vi "Add New State.vi"(7 "After State (Optional)":string, 8 "error in (no error)":errorcluster, 9 "State Name":string, 10 "Category (Optional)":string, 11 "JKI SM in":refnum<class "JKI SM.lvclass">) -> (0 "error out":errorcluster, 1 "New Frame Name":string, 3 "JKI SM out":refnum<class "JKI SM.lvclass">)   [LabVIEW 2020, in "JKI State Machine API.lvlib" / "JKI SM.lvclass"]
uses:
  JKI SM.lvclass
  JKI SM.lvclass/JKI SM.ctl
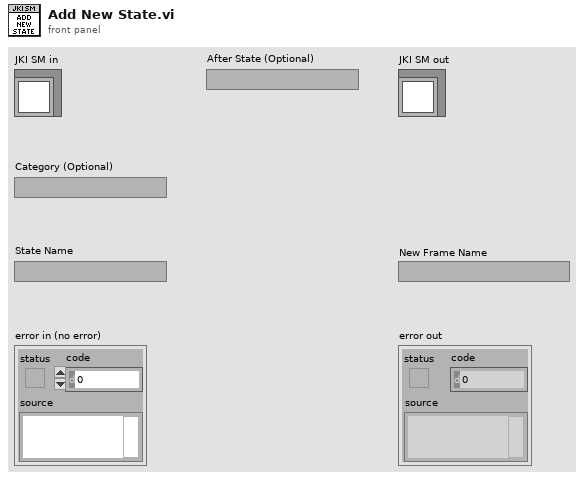
[diagram p1: front panel]
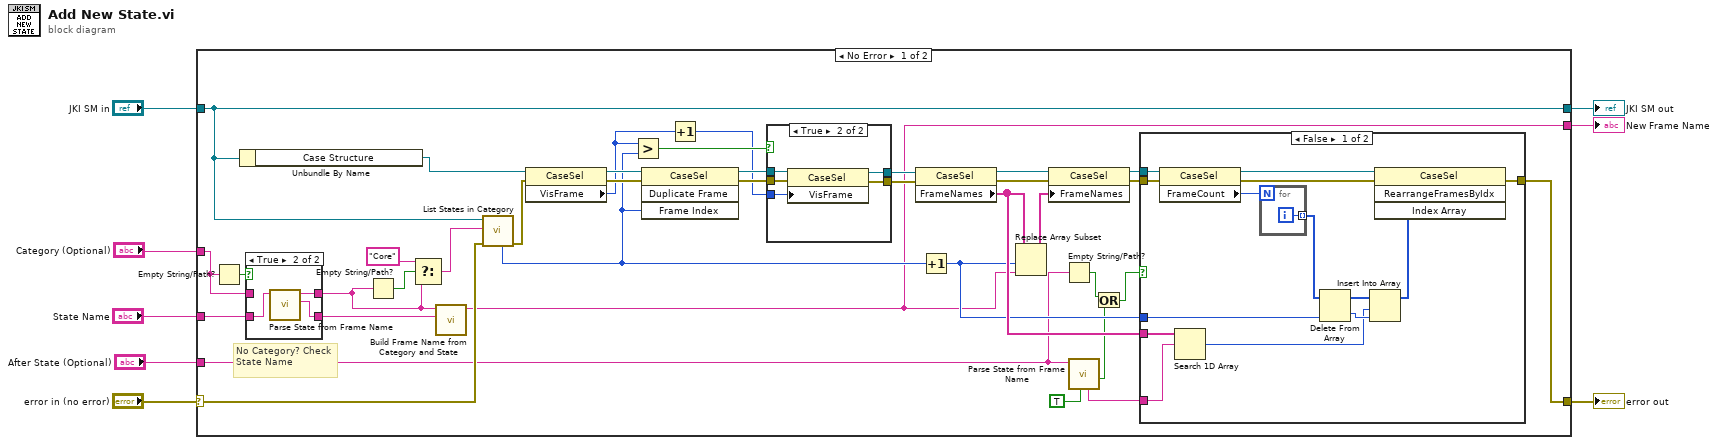
[diagram p0: block diagram]
diagram:
  n1 = case shown="No Error" "error in (no error)" {
    selector: "error in (no error)" -> [w42 w75]
    tunnel: [w16 w75] -> w7
    tunnel: [w20 w74] -> w5
    tunnel: "JKI SM in" -> [w20 w74]
    tunnel: "State Name" -> [w28 _]
    tunnel: "Category (Optional)" -> [w29 _]
    tunnel: "After State (Optional)" -> [w14 _]
    tunnel: [w9 _] -> w1
    frame No Error {
      # "No Category? Check State Name"
      n2 = Empty String/Path?(string/path=w29) -> (empty?=w30:bool)
      n3 = Unbundle By Name(w20) -> ("Case Structure"=w41:refnum<vi>)
      n4 = case shown="True" w30 {
        tunnel: w28 -> [w62 w66]
        tunnel: [w63 w65] -> w23
        tunnel: w29 -> [w63 _]
        tunnel: [w62 w64] -> w27
        frame False {
        }
        frame True {
          n5 = call "Parse State from Frame Name.vi"("Frame or State Name"=w66) -> ("State Name"=w64:string, "Category Name"=w65:string)  [unwired: 5 in, 4 out]
        }
      }
      n6 = Empty String/Path?(string/path=w23) -> (empty?=w25:bool)
      n7 = Select(t="Core" ("Category"), s=w25, f=w23) -> (s? t:f=w22:string)
      n8 = call "Build Frame Name from Category and State.vi"("State Name"=w27, "Category"=w23) -> ("Frame Name"=w9:string)  [unwired: 9 in]
      n9 = call "List States in Category.vi"("error in (no error)"=w42, "Category"=w22, "JKI SM in"=w20) -> ("error out"=w39:errorcluster, "Category Frame Index"=w26:i32)  [unwired: 4 in, 3 out]
      n10 = property class="CaseSel"(reference=w41, error in=w39) -> (reference out=w40:refnum<vi>, error out=w38:errorcluster, "VisFrame"=w33:u32)
      n11 = Greater?(x=w33, y=w26) -> (0:w32:bool)
      n12 = invoke class="CaseSel" method="Duplicate Frame"(reference=w40, error in=w38, "Frame Index"=w26) -> (reference out=w35:refnum<vi>, error out=w34:errorcluster)  [unwired: 1 in, 2 out]
      n13 = Increment(x=w33) -> (x+1=w31:u32)
      n14 = case shown="True" w32 {
        tunnel: [w68 w73] -> w37
        tunnel: [w67 w72] -> w36
        tunnel: w35 -> [w68 w71]
        tunnel: w34 -> [w67 w70]
        tunnel: w31 -> [_ w69]
        frame False {
        }
        frame True {
          n15 = property class="CaseSel"(reference=w71, error in=w70, "VisFrame"=w69) -> (reference out=w73:refnum<vi>, error out=w72:errorcluster)
        }
      }
      n16 = property class="CaseSel"(reference=w37, error in=w36) -> (reference out=w45:refnum<vi>, error out=w44:errorcluster, "FrameNames"=w21:string[])
      n17 = Increment(x=w26) -> (x+1=w18:i32)
      n18 = Replace Array Subset(array=w21, new element=w9, index=w18) -> (w43:string[])
      n19 = property class="CaseSel"(reference=w45, error in=w44, "FrameNames"=w43) -> (reference out=w19:refnum<vi>, error out=w17:errorcluster)
      n20 = Empty String/Path?(string/path=w14) -> (empty?=w12:bool)
      n21 = call "Parse State from Frame Name.vi"("Wrap in Quotes? (FALSE)"=TRUE, "Frame or State Name"=w14) -> ("is a Category Frame?"=w13:bool, "\"Category: State\" String"=w10:string)  [unwired: 4 in, 4 out]
      n22 = Or(x=w12, y=w13) -> (x .or. y?=w11:bool)
      n23 = case shown="False" w11 {
        tunnel: w21 -> [w54 _]
        tunnel: w19 -> [w52 _]
        tunnel: w18 -> [w51 _]
        tunnel: w17 -> [w48 w61]
        tunnel: [w49 w61] -> w16
        tunnel: w10 -> [w46 _]
        frame False {
          n24 = property class="CaseSel"(reference=w52, error in=w48) -> (reference out=w50:refnum<vi>, error out=w47:errorcluster, "FrameCount"=w55:i32)
          n25 = Search 1D Array(1D array=w54, element=w46) -> (index of element=w53:i32)  [unwired: 1 out]
          n26 = for {
            N: w55 -> [_]
            tunnel: [w60] -> w57 mode=indexing
            i -> [w60]
          }
          n27 = Delete From Array(array=w57, index=w51) -> (deleted portion=w58:i32, array with subset deleted=w59:i32[])  [unwired: 1 in]
          n28 = Insert Into Array(array=w59, index=w53, new element=w58) -> (w56:i32[])
          n29 = invoke class="CaseSel" method="RearrangeFramesByIdx"(reference=w50, error in=w47, "Index Array"=w56) -> (error out=w49:errorcluster)  [unwired: 1 in, 3 out]
        }
        frame True {
        }
      }
    }
    frame Error {
    }
  }
  "error out" <- w7
  "JKI SM out" <- w5
  "New Frame Name" <- w1
